vi "CSM - Interface Browser.vi"   [LabVIEW 2017]
doc: "Tools for browsing CSM module interfaces, allowing you to quickly view and search the API interfaces of CSM modules in the project."
uses:
  _ui/csm-ui-support.lvlib
types:
  T1 = enum32{"Bad", "Idle", "Run top level", "Running"}
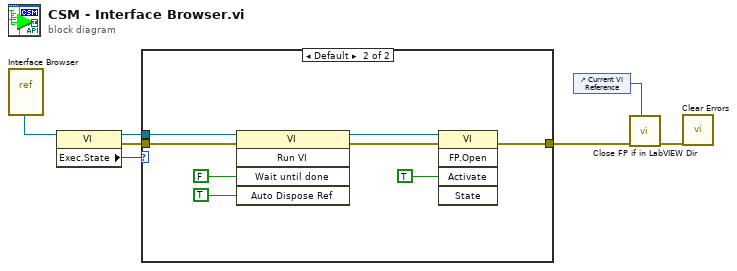
[diagram p0: block diagram]
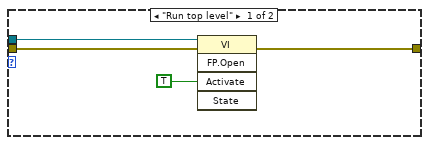
[diagram p2: hidden frame]
diagram:
  n1 = vi-ref "Interface Browser.vi"() -> (w5:refnum<vi>)
  n2 = property class="VI"(reference=w5) -> (reference out=w3:refnum<vi>, error out=w2:errorcluster, "Exec.State"=w4:T1)  [unwired: 1 in]
  n3 = case shown="Default" w4 {
    tunnel: w3 -> [w10 w19]
    tunnel: w2 -> [w11 w18]
    tunnel: [w8 w12] -> w1
    frame "Run top level" {
      n4 = invoke class="VI" method="FP.Open"(reference=w10, error in=w11, "Activate"=TRUE ("Activate?")) -> (error out=w8:errorcluster)  [unwired: 2 in, 4 out]
    }
    frame Default {
      n5 = invoke class="VI" method="Run VI"(reference=w19, error in=w18, "Wait until done"=FALSE ("Wait Until Done"), "Auto Dispose Ref"=TRUE ("Auto Dispose Reference")) -> (reference out=w15:refnum<vi>, error out=w14:errorcluster)  [unwired: 1 in, 3 out]
      n6 = invoke class="VI" method="FP.Open"(reference=w15, error in=w14, "Activate"=TRUE ("Activate?")) -> (error out=w12:errorcluster)  [unwired: 2 in, 4 out]
    }
  }
  n7 = control-ref of="Current VI Reference"() -> (w6:refnum<vi>)
  n8 = call "Close FP if in LabVIEW Dir.vi"("VI Refnum"=w6, "Error in"=w1) -> ("Error out"=w7:errorcluster)  [unwired: 9 in]
  n9 = call <vilib>:"Clear Errors.vi"("error in (no error)"=w7) -> ()  [unwired: 5 in, 2 out]
